vi "LabApp - Analog Output Simulator.vi"(6 "error in":errorcluster, 8 "Data In":dbl[](array[numeric]) format="%.2f") -> (0 "error out":errorcluster)   [LabVIEW 2021]
doc: "::: CalcExpress Toolkit :::\nCopyright (c) 2000-2026 Konstantin Shifershteyn. All rights reserved."
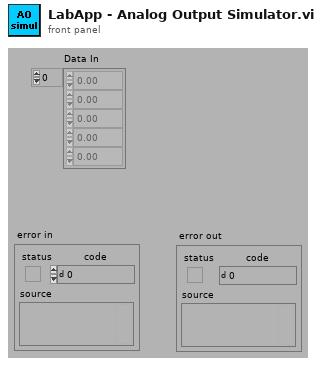
[diagram p1: front panel]
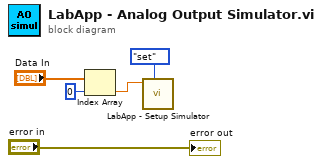
[diagram p0: block diagram]
diagram:
  n1 = Index Array(array="Data In", index=0) -> (element=w2:dbl)
  n2 = call "LabApp - Setup Simulator.vi"("cmd"=enum16{"init", "get", "set"}."set", "control"=w2) -> ()  [unwired: 6 in, 2 out]
  "error out" <- "error in"
